vi "VIH Utility - VISRV - Get Control Label & Caption.vi"(8 "error in":errorcluster, 11 "Ctrl Refnum":refnum<vi>) -> (0 "error out":errorcluster, 1 "Caption":string, 2 "Label":string, 3 "dup Ctrl Refnum":refnum<vi>, 4 "Has Caption":bool)   [LabVIEW 2014]
doc: "::: VI Helpeks :::\nCopyright (c) 2000-2026 Konstantin Shifershteyn. All rights reserved."
panel:
  # "VI Helpeks\nCopyright (c) 2012-2026 Konstantin Shifershteyn"
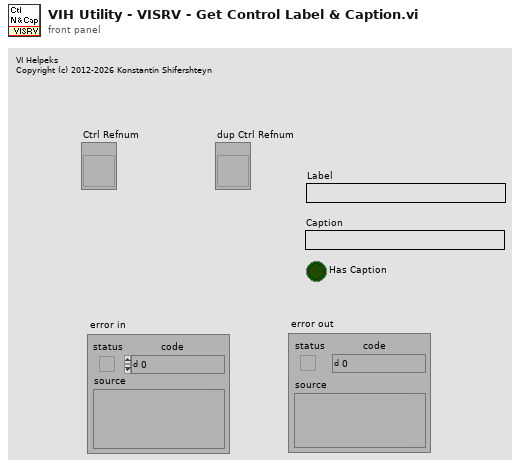
[diagram p1: front panel]
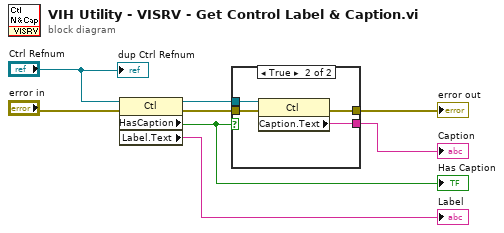
[diagram p0: block diagram]
diagram:
  n1 = property class="Ctl"(reference="Ctrl Refnum", error in="error in") -> (reference out=w8:refnum<vi>, error out=w7:errorcluster, "HasCaption"=w2:bool, "Label.Text"=→"Label":string)
  "Has Caption" <- w2
  n2 = case shown="True" w2 {
    tunnel: w8 -> [_ w13]
    tunnel: w7 -> [w9 w12]
    tunnel: [_ w11] -> w3
    tunnel: [w9 w10] -> w4
    frame False {
    }
    frame True {
      n3 = property class="Ctl"(reference=w13, error in=w12) -> (error out=w10:errorcluster, "Caption.Text"=w11:string)  [unwired: 1 out]
    }
  }
  "error out" <- w4
  "Caption" <- w3
  "dup Ctrl Refnum" <- "Ctrl Refnum"
